vi "PicoScope2000aRunBlock.vi"(7 "Acquisition Settings":T1 {"postTriggerSamples" format="%_6p"; "preTriggerSamples" format="%_6p"}, 8 "error in (no error)":errorcluster, 11 "handle in":i16) -> (0 "error out":errorcluster, 3 "handle out":i16, 4 "timeIndisposedMs":dbl, 6 "Total Requested Samples":u64)   [LabVIEW 2009]
doc: "Calls RunBlock"
uses:
  ps2000a.dll
  shared/Acquisition Settings.ctl
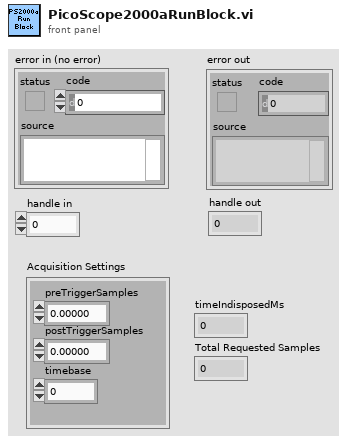
[diagram p1: front panel]
types:
  T1 = typedef "Acquisition Settings.ctl" = cluster{"preTriggerSamples":u64, "postTriggerSamples":u64, "timebase":u32}
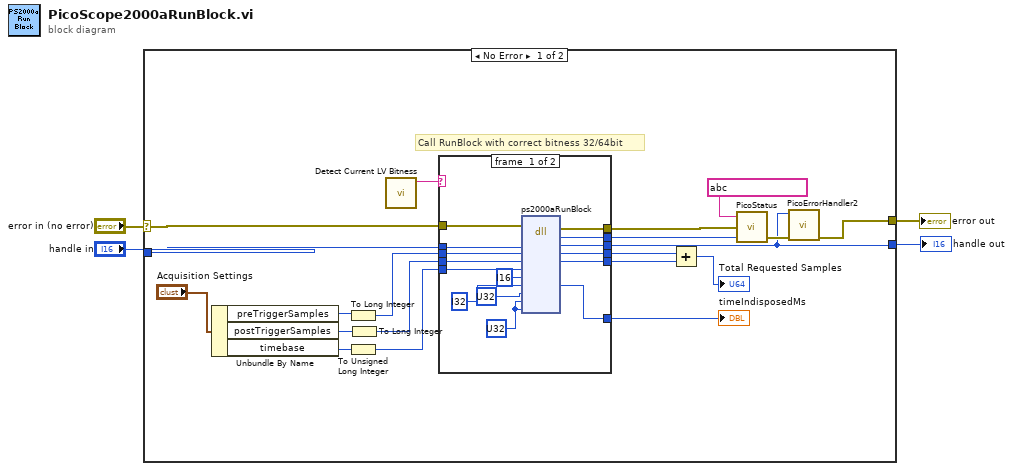
[diagram p0: block diagram]
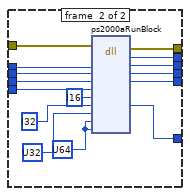
[diagram p2: hidden frame]
diagram:
  n1 = case shown="No Error" "error in (no error)" {
    selector: "error in (no error)" -> [w18 w56]
    tunnel: [w14 w56] -> w2
    tunnel: "handle in" -> [w17 w55]
    tunnel: [w13 w55] -> w3
    frame #0 {
      # "Call RunBlock with correct bitness 32/64bit"
      n2 = Unbundle By Name("Acquisition Settings") -> ("preTriggerSamples"=w10:u64, "postTriggerSamples"=w8:u64, "timebase"=w9:u32)
      n3 = To Long Integer(number=w10) -> (32bit integer=w7:i32)
      n4 = To Unsigned Long Integer(number=w9) -> (unsigned 32bit integer=w5:u32)
      n5 = To Long Integer(number=w8) -> (32bit integer=w6:i32)
      n6 = call "Detect Current LV Bitness.vi"() -> ("bitness"=w15:string)  [unwired: 11 in]
      n7 = case shown="\"64\"" w15 {
        tunnel: [w39 w54] -> w24
        tunnel: [w38 w53] -> w23
        tunnel: [w37 w52] -> w21
        tunnel: [w36 w51] -> w20
        tunnel: w18 -> [w35 w50]
        tunnel: w17 -> [w34 w49]
        tunnel: w7 -> [w32 w47]
        tunnel: w6 -> [w31 w46]
        tunnel: w5 -> [w30 w45]
        tunnel: [w29 w44] -> w13
        tunnel: [w26 w42] -> w12
        frame #0 {
          w28 = u32 ? ("pParameter")
          n8 = dll-call lib="ps2000a.dll" fn="ps2000aRunBlock" ("ps3000.dll:_ps3000_open_unit@0")(error in=w35, "handle"=w34, "noOfPreTriggerSamples"=w32, "noOfPostTriggerSamples"=w31, "timebase"=w30, "oversample"=i16 ?, "timeIndisposedMs"=i32 ? ("pParameter"), "segmentIndex"=u32 ?, "lpReady"=w28, "pParameter"=w28) -> (error out=w36:errorcluster, "PICO_STATUS"=w37:u32, "handle"=w29:i16, "noOfPreTriggerSamples"=w39:i32, "noOfPostTriggerSamples"=w38:i32, "timeIndisposedMs"=w26:i32)  [unwired: 7 in, 1 out]
        }
        frame #1 {
          w43 = u64 ? ("pParameter")
          n9 = dll-call lib="ps2000a.dll" fn="ps2000aRunBlock" ("ps3000.dll:_ps3000_open_unit@0")(error in=w50, "handle"=w49, "noOfPreTriggerSamples"=w47, "noOfPostTriggerSamples"=w46, "timebase"=w45, "oversample"=i16 ?, "timeIndisposedMs"=i32 ? ("pParameter"), "segmentIndex"=u32 ?, "lpReady"=w43, "pParameter"=w43) -> (error out=w51:errorcluster, "PICO_STATUS"=w52:u32, "handle"=w44:i16, "noOfPreTriggerSamples"=w54:i32, "noOfPostTriggerSamples"=w53:i32, "timeIndisposedMs"=w42:i32)  [unwired: 7 in, 1 out]
        }
      }
      "timeIndisposedMs" <- w12
      n10 = Add(x=w24, y=w23) -> (x+y=→"Total Requested Samples":i32)
      n11 = call "PicoStatus.vi"("PICO STATUS"=w21, "error in"=w20, "source"=string ?) -> ("error out"=w16:errorcluster)
      n12 = call "PicoErrorHandler2.vi"("error in (no error)"=w16, "handle In"=w13) -> ("error out"=w14:errorcluster)  [unwired: 9 in]
    }
    frame #1 {
    }
  }
  "error out" <- w2
  "handle out" <- w3
